vi "plotting_subvi_chirp__ac85fa7053.vi"(6 "commanded strain":dbl[](array[numeric]), 9 "real strain (-)":dbl[](array[numeric]), 10 "iteration":dbl, 11 "current":dbl[](array[numeric])) -> (2 "Mixed Signal Graph":dynamicdata(graph) caption="Commanded and Actual Strain vs Current", 3 "Lissajou":cluster{dbl[], dbl[]}(graph))   [LabVIEW 2023]
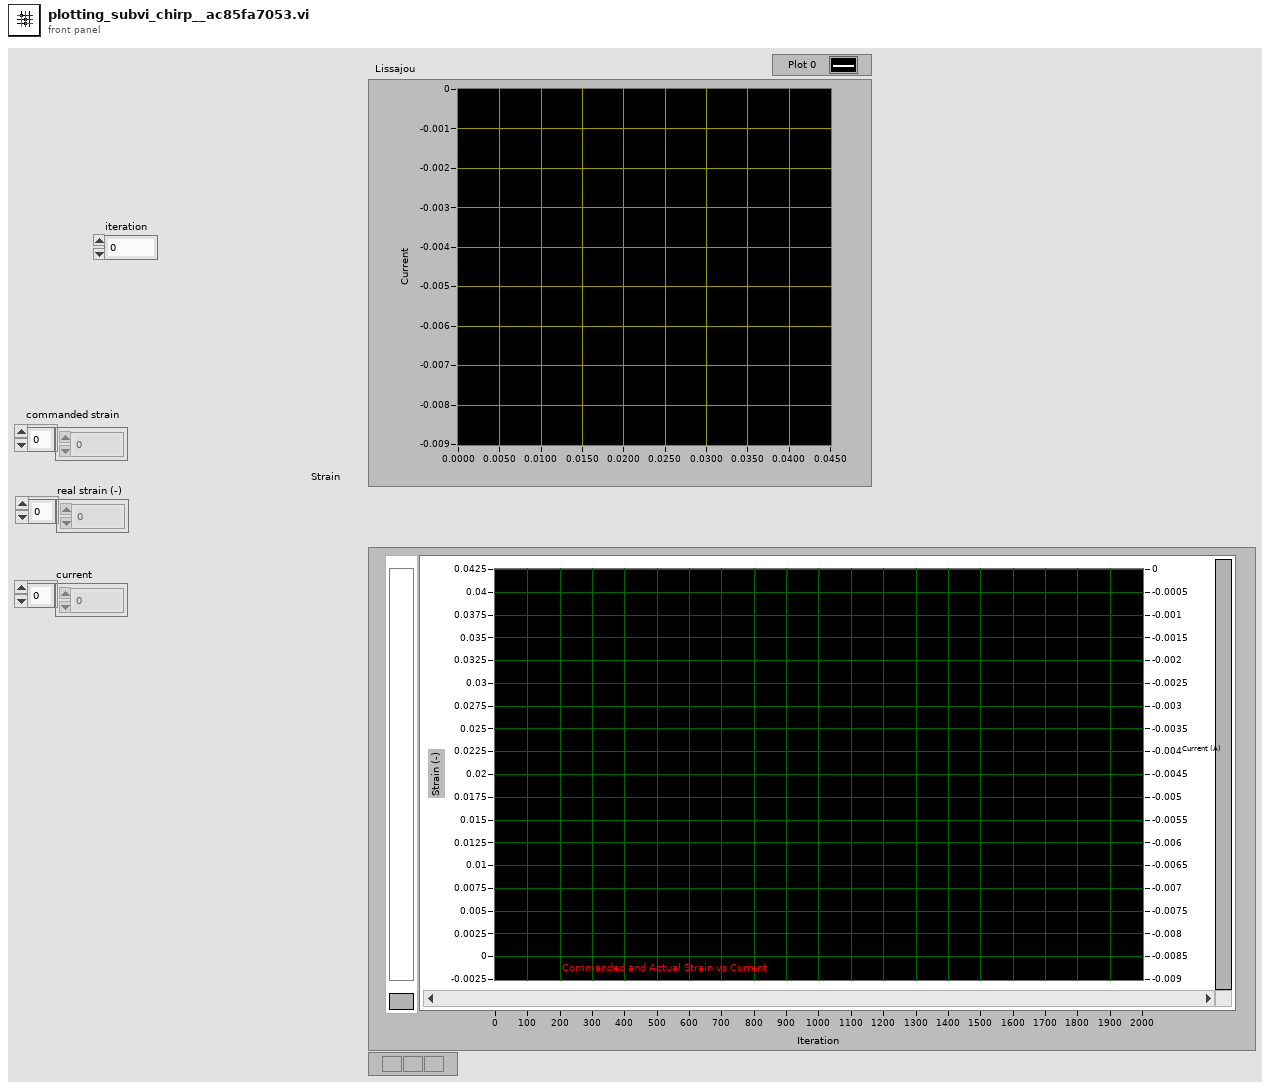
[diagram p1: front panel]
types:
  T1 = cluster{"real strain (-)":dbl[], "current":dbl[]}
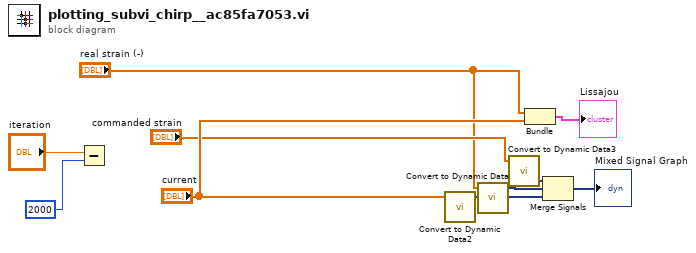
[diagram p0: block diagram]
diagram:
  n1 = Subtract(x="iteration", y=2000 ("length")) -> ()  [unwired: 1 out]
  n2 = call "Convert to Dynamic Data2"("Array"="current") -> ("Dynamic Data Type"=w8:dynamicdata)  [unwired: 3 in]
  n3 = call "Convert to Dynamic Data"("Array"="real strain (-)") -> ("Dynamic Data Type"=w7:dynamicdata)  [unwired: 3 in]
  n4 = call "Convert to Dynamic Data3"("Array"="commanded strain") -> ("Dynamic Data Type"=w10:dynamicdata)  [unwired: 3 in]
  n5 = Bundle("real strain (-)"="real strain (-)", "current"="current") -> (→"Lissajou":T1)  [unwired: 1 in]
  n6 = Merge Signals(w10, w7, w8) -> (→"Mixed Signal Graph":dynamicdata)
